vi "Dashboard Main.vi"() -> ()   [LabVIEW 2017]
uses:
  <vilib>/Rock Robotics/WPI/DriverStation/WPI_DriverStationAllianceInfo.ctl
  <vilib>/Utility/miscctls.llb/LVRowAndColumnTypeDef.ctl
  <vilib>/event_ctls.llb/eventvkey.ctl
  <vilib>/Rock Robotics/Network Tables/NT Read Numeric Array.vi
  <vilib>/Rock Robotics/WPI/Dashboard/WPI_DashboardLogging Global.vi
  <vilib>/Rock Robotics/Network Tables/NT Write Numeric Array.vi
  <vilib>/Rock Robotics/Network Tables/NT Read Boolean.vi
  <vilib>/Rock Robotics/Network Tables/NT Write Boolean.vi
panel:
  out "NT Connection":bool=TRUE
  in  "Camera Settings Right":T1={"Frame Rate"=15, "Compression"=30, "Size"=1, "DB Camera Config"=FALSE} {"Frame Rate" scale=1.0..30.0; "Compression" scale=100.0..-1.0; "Size" items=["640x480", "320x240", "160x120"]}
  in  "Camera Name Right":string(combo)="No Camera Selection"
  out "Camera Info":cluster{"Mbps LED":bool, "Mbps":dbl, "fps":dbl}={"Mbps LED"=FALSE, "Mbps"=0.17652911574406902, "fps"=9.930486593843098} {"fps" format="%#.1g"; "Mbps" format="%#.1g"}
  in  "Camera Settings":T1={"Frame Rate"=10, "Compression"=66, "Size"=2, "DB Camera Config"=FALSE} {"Frame Rate" scale=1.0..30.0; "Compression" scale=100.0..-1.0; "Size" items=["640x480", "320x240", "160x120"]}
  in  "TCP":refnum<k5>
  in  "Rec Mode":enum32{"Stop", "Record", "Playback"}(radio)
  out "Robot IP":string="10.17.12.2"
  out "Image Message":string="Timeout in Camera Communications"
  in  "Dashboard Tab":T2(tab)
  out "PixyX":dbl(slide)=26.65616755102041 scale=0.0..320.0
  in  "Reset":bool
  out "FastMode":bool
  out "ToggleMode":bool
  out "HasCube":bool
  out "Mode":T3(ring)
  out "Gyro":dbl(knob)=-172.57 scale=-180.0..180.0
  out "Elevator":dbl(slide)=5.727272727272727 scale=-10.0..80.0
  out "LeftEncoder":dbl=817.74403425
  out "RightEncoder":dbl=362.091195
  out "Ultrasonic":dbl(slide)=26.65616755102041 scale=0.0..60.0
  out "Bottom":bool
  out "Top":bool
  out "Camera Image Right":T4(plugin-control)
  in  "DB/String 9":string
  in  "DB/String 8":string
  in  "DB/String 7":string
  in  "DB/String 6":string
  in  "DB/String 5":string
  in  "DB/String 4":string
  in  "DB/String 3":string
  in  "DB/String 2":string
  in  "DB/String 1":string
  in  "DB/String 0":string
  in  "DB/Slider 0":dbl(slide) scale=0.0..5.0
  in  "DB/Slider 1":dbl(slide) scale=0.0..5.0
  in  "DB/Slider 2":dbl(slide) scale=0.0..5.0
  in  "DB/Slider 3":dbl(slide) scale=0.0..5.0
  out "DB/LED 3":bool
  out "DB/LED 2":bool
  out "DB/LED 1":bool
  out "DB/LED 0":bool
  in  "DB/Button 3":bool
  in  "DB/Button 2":bool
  in  "DB/Button 1":bool
  in  "DB/Button 0":bool caption="New Name"
  in  "RR Delay":dbl
  in  "LR Delay":dbl
  in  "LL Delay":dbl
  in  "RRAction2":dbl
  in  "LRAction2":dbl
  in  "LLAction2":dbl
  in  "RRAction1":dbl
  in  "LRAction1":dbl
  in  "LLAction1":dbl
  in  "NotPurePursuit":bool
  in  "Battery Number":string
  out "?":bool=TRUE
  out "Opponent Right Switch":bool
  out "Center Left Scale":bool=TRUE
  out "Center Right Scale":bool
  out "Our Left Team Switch":bool=TRUE
  out "Our Right Team Switch":bool
  in  "Position":u32=3
  in  "RLAction1":dbl
  in  "RLAction2":dbl
  in  "RL Delay":dbl
  in  "Test Slider":dbl(slide) scale=0.0..100.0 scale format="%#_3g"
  in  "On/Off":bool caption="Solenoid"
  in  "Test Name":u16(ring) items=["Select the test to run..."]
  in  "Test Tree":string(tree)
  in  "Motor":cluster{"Value":dbl, "Enable":bool} {"Value" scale=-1.0..1.0 scale format="%#_3g"}
  out "Progress":T5 {"Test Progress" scale=0.0..100.0}
  in  "Rev/Fwd":cluster{"Forward":bool, "Reverse":bool}
  in  "Test Ring":u16(ring) items=["Monochrome", "Color"]
  out "Cmd Status":string
  in  "Execute Command":bool
  in  "Command Params":string[][](table)
  in  "Command Selection":i32(listbox)
  in  "CheckList":i32(listbox)
  out "Tree":string(tree)
  out "Camera Image":T4(plugin-control)
  in  "Camera Name":string(combo)="Camera"
  # "Don't use this row"
  # "HW"
  # "HW"
  # "Switch/Scale Positions"
  # "1Cube"
  # "2Cube"
  # "Delay"
  # "Left"
  # "Left"
  # "Right"
  # "Left"
  # "Left"
  # "Right"
  # "Right"
  # "Right"
  # "Action Key:\n0 = Do Nothing\n1 = Go Switch\n2 = Go Scale"
  # "1"
  # "2"
  # "3"
  # "4"
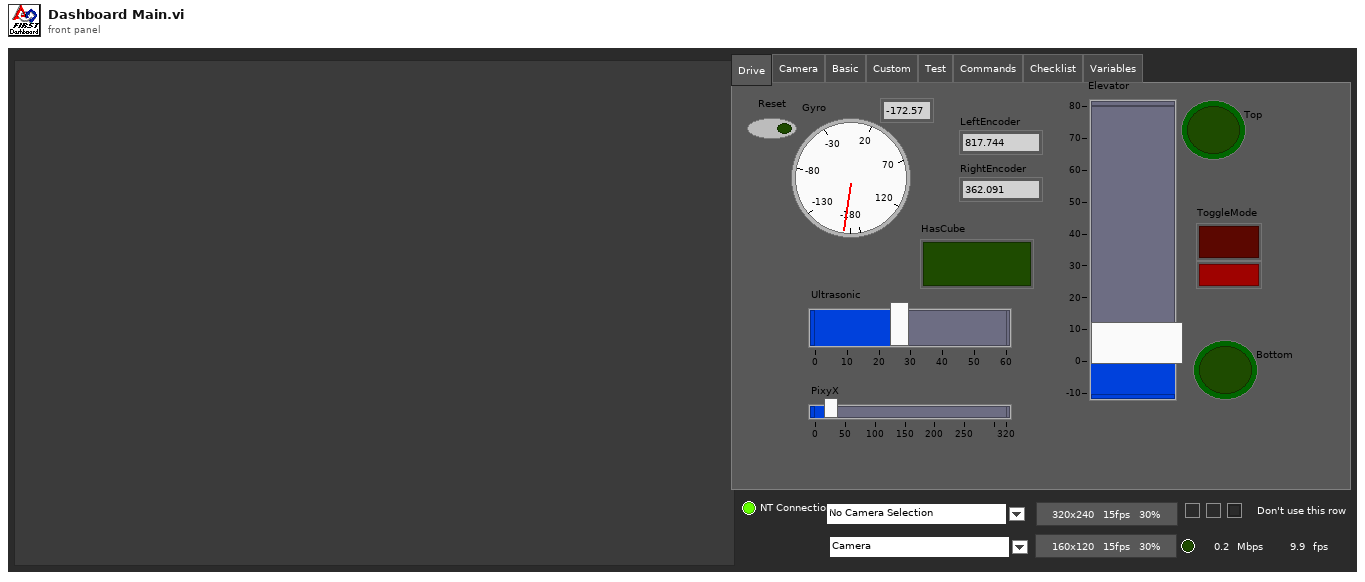
[diagram p1: front panel]
types:
  T1 = cluster{"Frame Rate":i32, "Compression":i32, "Size":u16, "DB Camera Config":bool}
  T2 = enum32{"Drive", "Camera", "Basic", "Custom", "Test", "Commands", "Checklist", "Variables"}
  T3 = enum8{"Tele-Op Disabled", "Tele-Op Enabled", "Auto Disabled", "Auto Enabled", "Test Disabled", "Test Enabled", "Disconnected", "No Code", "E-Stop"}
  T4 = typedef "IMAQ Image.ctl" = refnum<image>
  T5 = cluster{"Test Progress":u8, "Test Progress Text":string}
  T6 = cluster{"Save Path":path, "Interval (s)":dbl, "Keep":i32}
  T7 = typedef "Image Type" = u32
  T8 = cluster{"IDs":cluster{"RPC field ID":u16, "Unique ID":u16}, "String":string}
  T9 = cluster{"Error Strings":string, "Disable Counts":cluster{u16, u16}, "Rail Faults":cluster{u16, u16, u16}, "Robot IP":string, "DB Mode":u8, "Event Info":cluster{"Name":string, "Type":u8, "Number":u16, "Replay":u8}}
  T10 = cluster{"Storage":cluster{"Disk Free":u64, "RAM Block":u32, "RAM free":u32}, "CPU Utilization":cluster{"CPU % ISR":sgl, "CPU % Time Crit":sgl, "CPU % Timed Str":sgl, "CPU % High":sgl, "CPU % Above":sgl, "CPU % Normal":sgl, "CPU % Low":sgl}, "CAN":cluster{"% Bus Utilization":sgl, "Bus Off Cnt":u32, "TX_FIFO Full Cnt":u32, "Receive Error Cnt":u8, "Transmit Error Cnt":u8}, "HID":cluster{"HID Outputs":u32, "Rumble Low":u16, "Rumble High":u16}[]}
  T11 = cluster{"Status bits":cluster{"Test Mode":bool, "Autonomous":bool, "Enabled":bool, "Code Start":bool, "Brownout":bool, "Reserved 2":bool, "Reserved 3":bool, "E-Stop":bool}, "Code Trace":cluster{"Disabled":bool, "TeleOp":bool, "Auto":bool, "Test":bool}, "Controller Type":enum16{"unknown", "cRIO", "roboRio"}, "Code?":enum16{"unknown", "noCode", "code"}, "Battery V":dbl}
  T12 = cluster{"Control Bits":cluster{"TestMode":bool, "Autonomous":bool, "Enabled":bool, "FMS Present":bool, bool, bool, bool, "E-Stop":bool}, "Team Station ":u8, "Countdown":sgl, "Joystick Values":cluster{"Axes":dbl[], "Buttons":bool[], "POVs":i16[]}[]}
  T13 = cluster{"Axes":dbl[], "Buttons":bool[], "POVs":i16[]}[]
  T14 = cluster{"Axes":dbl[], "Buttons":bool[], "POVs":i16[]}
  T15 = cluster{"Camera Image":refnum<vi>, "Dashboard Tab":refnum<vi>, "Rec Mode":refnum<vi>, "Test Slider":refnum<vi>, "On/Off ":refnum<vi>, "Test Ring":refnum<vi>, "Rev/Fwd":refnum<vi>, "Test Name":refnum<vi>, "Motor":refnum<vi>, "Progress":refnum<vi>, "CheckList":refnum<vi>, "Tree":refnum<vi>, "Test Tree":refnum<vi>, "Command Params":refnum<vi>, "Command Selection":refnum<vi>, "Execute Command":refnum<vi>, "Cmd Status":refnum<vi>, "Camera Settings":refnum<vi>, "Camera Name":refnum<vi>, "Camera Info":refnum<vi>, "Camera Settings Right":refnum<vi>, "Camera Name Right":refnum<vi>, "Camera Image Right":refnum<vi>}
  T16 = cluster{"Camera Name":string, string, "Saved DB Images Info":cluster{"Save Path":path, "Interval (s)":dbl, "Keep":i32}}
  T17 = cluster{"Camera Name Right":string, string, "Saved DB Images Info":cluster{"Save Path":path, "Interval (s)":dbl, "Keep":i32}}
  T18 = typedef "WPI_DriverStationAllianceInfo.ctl" = enum16{"Red", "Blue", "Invalid"}
  T19 = cluster{"Operation":enum16{"Update", "Clear"}, "Color Box":u32}[]
  T20 = typedef "eventvkey.ctl" = enum16{"ASCII", "Enter", "Return", "Shift", "Ctrl", "Alt", "Cmd", "Opt", "Caps", "NumLock", "Clear", "Break", "Up", "Down", "Left", "Right", "Insert", "Delete", "Home", "End", "PageUp", "PageDown", "Escape", "Help", "Pause", "ScrollLock", "F1", "F2", "F3", "F4", "F5", "F6", "F7", "F8", "F9", "F10", "F11", "F12", "F13", "F14", "F15", "F16", "F17", "F18", "F19", "F20", "F21", "F22", "F23", "F24", "Play", "VolumeUp", "VolumeDown", "Mute", "Two Byte Char"}
  T21 = cluster{"Image Size":bool, "Image Type":bool, "Pixel Value":bool, "ROI Information":bool, "Zoom Factor":bool}
  T22 = cluster{"Operation":enum16{"Update", "Clear"}, "Color Box":u32}
  T23 = typedef "LVRowAndColumnTypeDef.ctl" = cluster{"Row":i32, "Column":i32}
  T24 = cluster{"Shift":bool, "Ctrl":bool, "Alt":bool, "Cmd":bool, "Opt":bool}
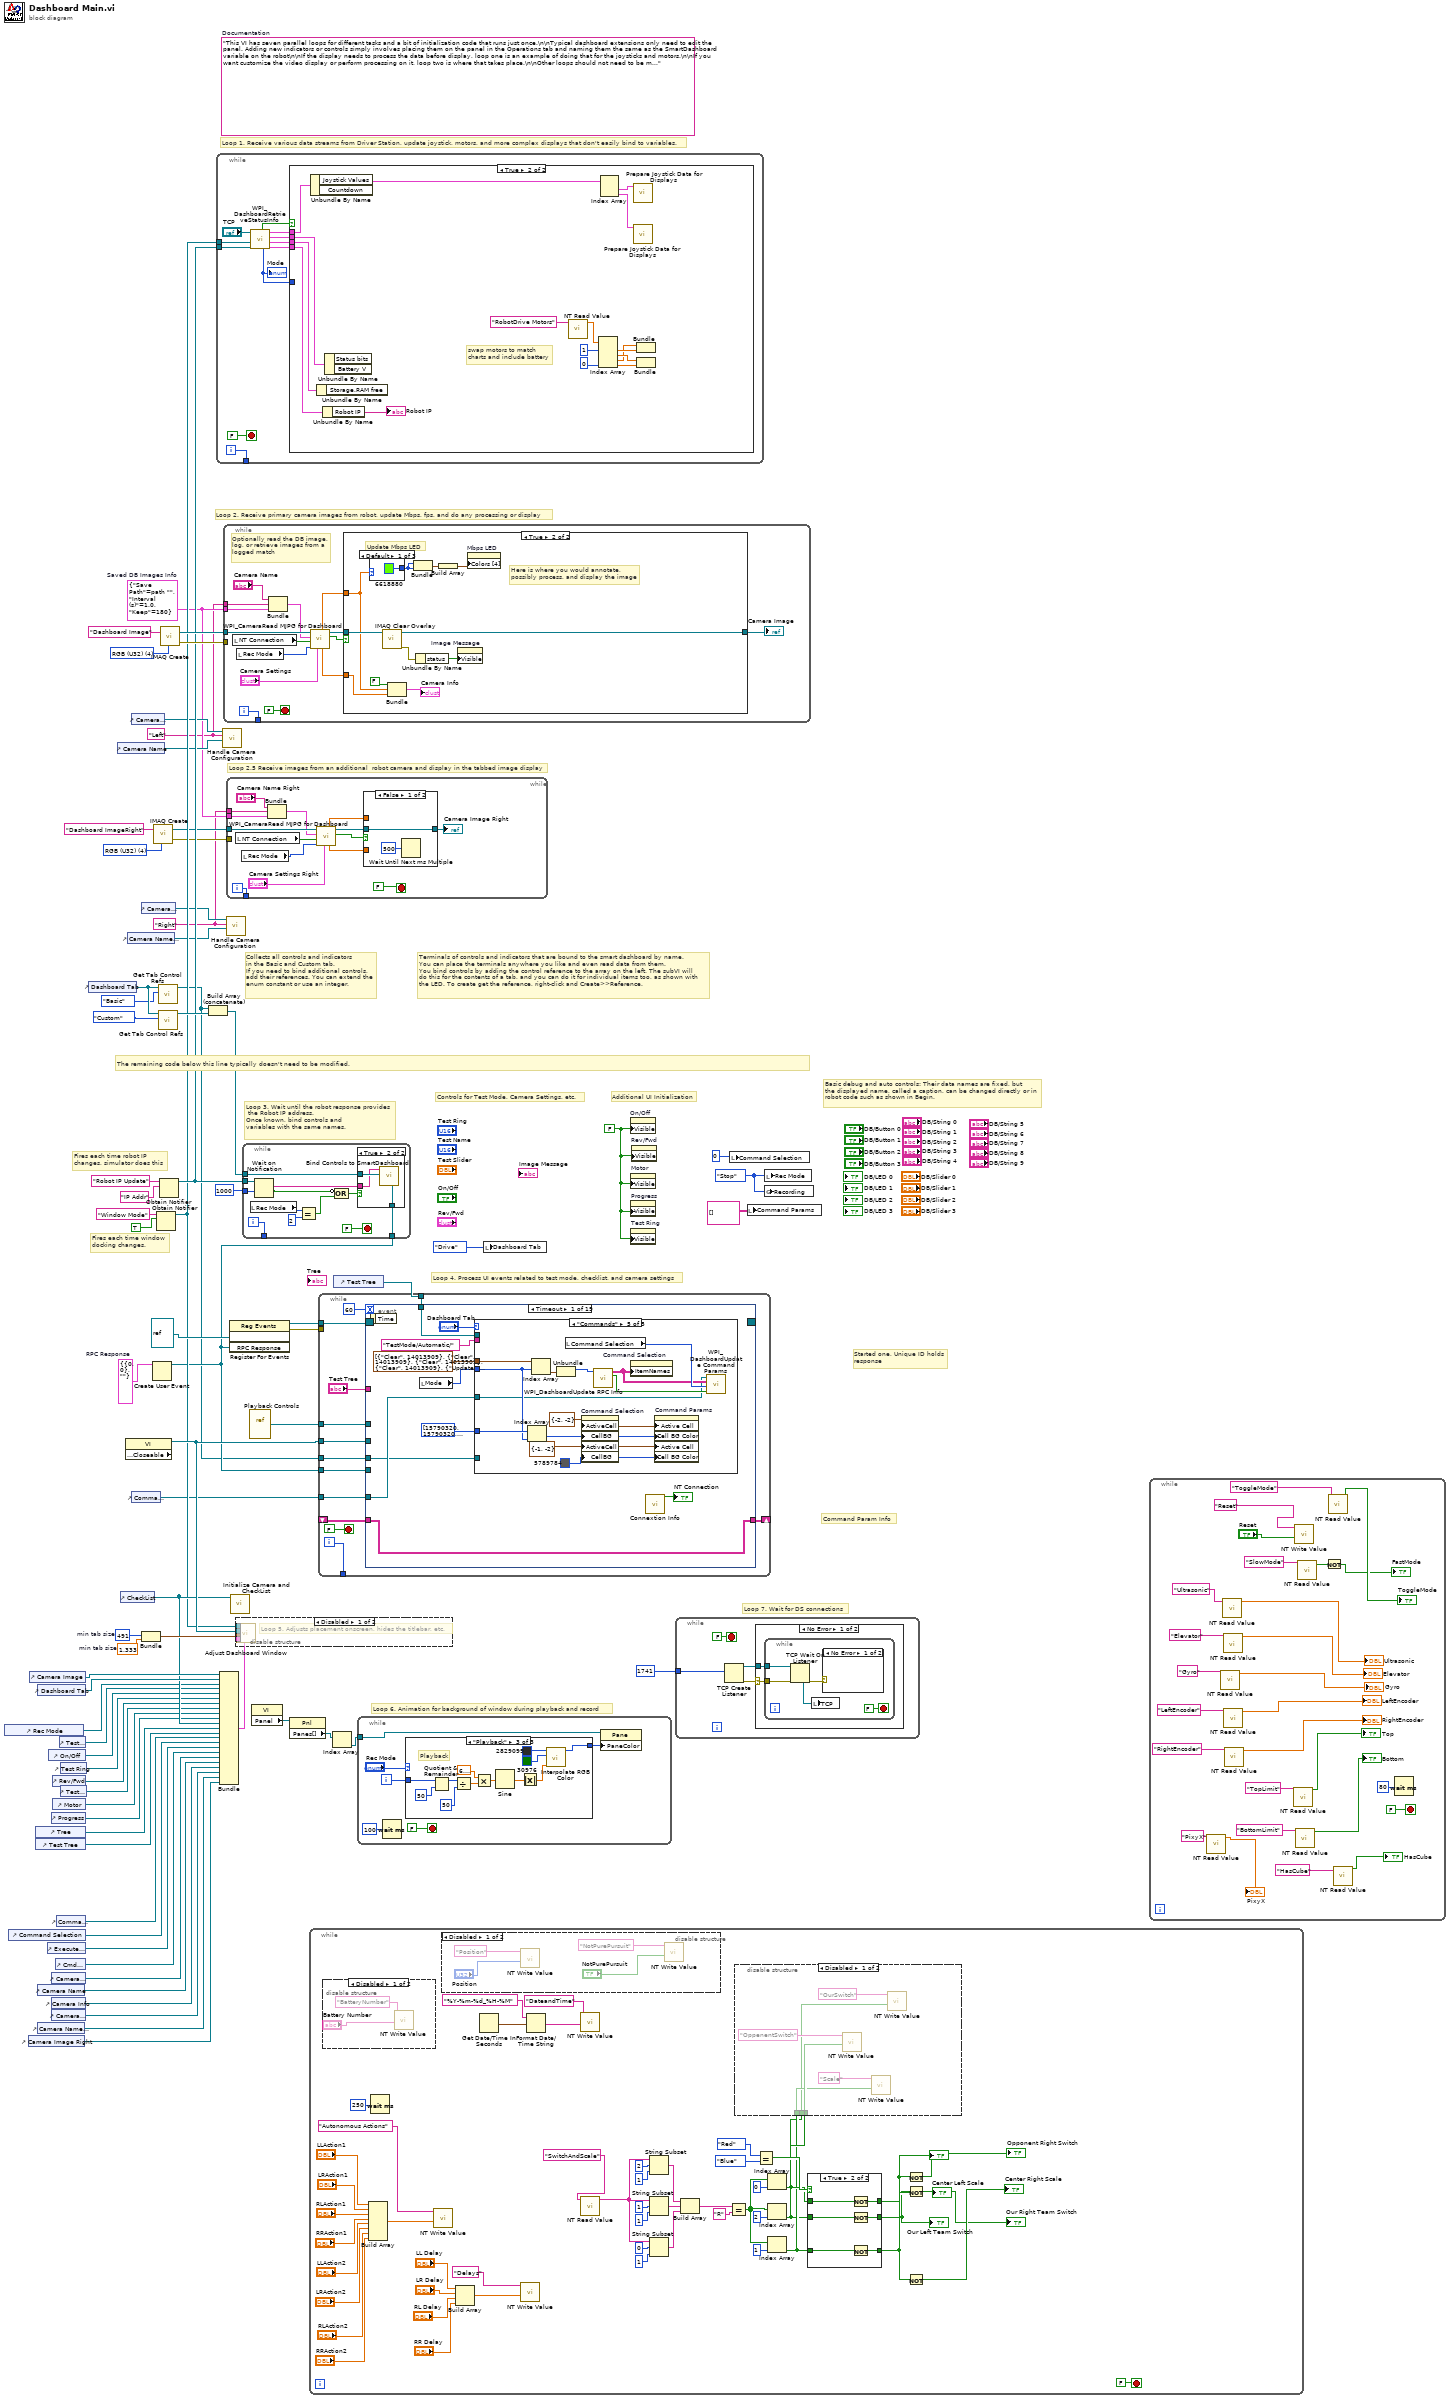
[diagram p0: block diagram]
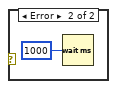
[diagram p8: hidden frame]
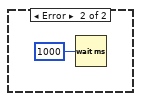
[diagram p9: hidden frame]
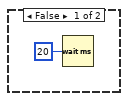
[diagram p10: hidden frame]
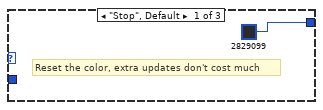
[diagram p11: hidden frame]
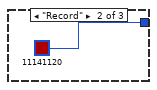
[diagram p12: hidden frame]
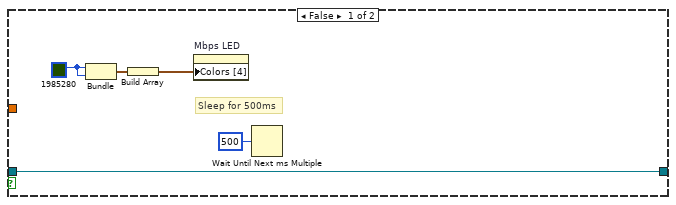
[diagram p14: hidden frame]
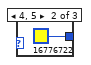
[diagram p15: hidden frame]
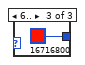
[diagram p16: hidden frame]
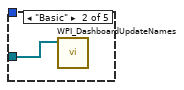
[diagram p18: hidden frame]
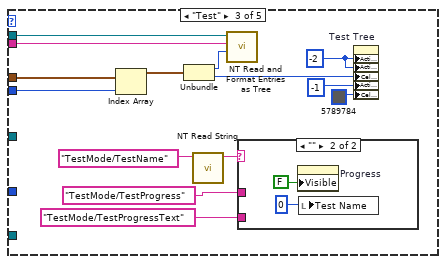
[diagram p19: hidden frame]
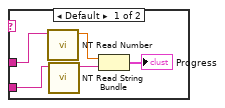
[diagram p20: hidden frame]
diagram:
  w4 = T6 {"Save Path"=path "", "Interval (s)"=1.0, "Keep"=180}  # Saved DB Images Info
  w3 = "Right"
  w2 = "Left"
  w14 = T7 4 items=["Grayscale (U8)", "Grayscale (I16)", "Grayscale (SGL)", "Complex (CSG)", "RGB (U32)", "HSL (U32)", "RGB (U64)"] ("Image Type")
  w28 = T8 {"IDs"={"RPC field ID"=0, "Unique ID"=0}, "String"=""}  # RPC Response
  w49 = 491  # min tab size
  w48 = 1.333  # min tab size
  w56 = enum32{"Stop", "Record", "Playback"}."Stop" ("Rec Mode")
  w34 = FALSE ("Visible")
  (unwired) "This VI has seven parallel loops for different tasks and a bit of initialization code that runs just once.\n\nTypical dashboard extensions only need to edit the panel. Adding new indicators or controls simply involves placing them on the panel in the Operations tab and naming them the same as the SmartDashboard variable on the robot\n\nIf the display needs to process the data before display, loop one is an example of doing that for the joysticks and motors.\n\nIf you want customize the video display or perform processing on it, loop two is where that takes place.\n\nOther loops should not need to be modified. They are pretty standard, and document the task they perform."  # Documentation
  w73 = T7 4 items=["Grayscale (U8)", "Grayscale (I16)", "Grayscale (SGL)", "Complex (CSG)", "RGB (U32)", "HSL (U32)", "RGB (U64)"] ("Image Type")
  # "Loop 2.5 Receive images from an additional  robot camera and display in the tabbed image display"
  # "Command Param Info"
  # "Started one, Unique ID holds\nresponse"
  # "Loop 7. Wait for DS connections"
  # "Basic debug and auto controls: Their data names are fixed, but\nthe displayed name, called a caption, can be changed directly or in\nrobot code such as shown in Begin."
  # "Controls for Test Mode, Camera Settings, etc."
  # "Additional UI Initialization"
  # "Loop 6. Animation for background of window during playback and record"
  # "Fires each time robot IP\nchanges, simulator does this"
  # "Fires each time window\ndocking changes."
  # "Collects all controls and indicators\nin the Basic and Custom tab.\nIf you need to bind additional controls,\nadd their references. You can extend the\nenum constant or use an integer."
  # "The remaining code below this line typically doesn't need to be modified."
  # "Loop 4. Process UI events related to test mode, checklist, and camera settings"
  # "Terminals of controls and indicators that are bound to the smart dashboard by name.\nYou can place the terminals anywhere you like and even read data from them.\nYou bind controls by adding the control reference to the array on the left. The subVI will\ndo this for the contents of a tab, and you can do it for individual items too, as shown with\nthe LED. To create get the reference, right-click and Create>>Reference."
  # "Loop 3. Wait until the robot response provides\n the Robot IP address.\nOnce known, bind controls and\nvariables with the same names."
  # "Loop 1. Receive various data streams from Driver Station, update joystick, motors, and more complex displays that don't easily bind to variables."
  # "Loop 2. Receive primary camera images from robot, update Mbps, fps, and do any processing or display"
  n1 = control-ref of="Rec Mode"() -> (w40:refnum<vi>)
  n2 = control-ref of="Command Selection"() -> (w27:refnum<vi>)
  n3 = control-ref of="Camera Image Right"() -> (w7:refnum<vi>)
  n4 = control-ref of="Camera Image"() -> (w51:refnum<vi>)
  n5 = control-ref of="Tree"() -> (w44:refnum<vi>)
  n6 = control-ref of="Test Tree"() -> (w43:refnum<vi>)
  n7 = control-ref of="Dashboard Tab"() -> (w50:refnum<vi>)
  n8 = control-ref of="Camera Name"() -> (w18:refnum<vi>)
  n9 = control-ref of="Camera Name Right"() -> (w8:refnum<vi>)
  n10 = control-ref of="Execute Command"() -> (w29:refnum<vi>)
  n11 = control-ref of="On/Off"() -> (w38:refnum<vi>)
  n12 = control-ref of="Progress"() -> (w35:refnum<vi>)
  n13 = control-ref of="Camera Settings"() -> (w19:refnum<vi>)
  n14 = control-ref of="Camera Info"() -> (w17:refnum<vi>)
  n15 = control-ref of="Camera Settings Right"() -> (w9:refnum<vi>)
  n16 = control-ref of="Rev/Fwd"() -> (w36:refnum<vi>)
  n17 = control-ref of="Motor"() -> (w41:refnum<vi>)
  n18 = control-ref of="Cmd Status"() -> (w23:refnum<vi>)
  n19 = control-ref of="Command Params"() -> (w30:refnum<vi>)
  n20 = control-ref of="Test Slider"() -> (w39:refnum<vi>)
  n21 = control-ref of="Test Ring"() -> (w37:refnum<vi>)
  n22 = control-ref of="Test Name"() -> (w42:refnum<vi>)
  n23 = control-ref of="Dashboard Tab"() -> (w54:refnum<vi>)
  n24 = control-ref of="Camera Name"() -> (w20:refnum<vi>)
  n25 = control-ref of="CheckList"() -> (w45:refnum<vi>)
  n26 = property class="VI" props=["Front Panel.Closeable"]() -> (reference out=w55:refnum<vi>)  [unwired: 2 in, 2 out]
  n27 = control-ref of="Camera Name Right"() -> (w10:refnum<vi>)
  n28 = control-ref of="Camera Settings"() -> (w21:refnum<vi>)
  n29 = control-ref of="Command Params"() -> (w22:refnum<vi>)
  n30 = control-ref of="Camera Settings Right"() -> (w11:refnum<vi>)
  n31 = Bundle("min tab size"=w49, "min tab size"=w48) -> (w47:cluster{"min tab size":i32, "min tab size":dbl})  [unwired: 1 in]
  n32 = Create User Event(user event datatype=w28) -> (user event=w24:refnum<user-event>)  [unwired: 1 in, 1 out]
  n33 = call "IMAQ Create"("Image Name"="Dashboard ImageRight", "Image Type"=w14) -> ("New Image"=w13:T4, "error out"=w12:errorcluster)  [unwired: 2 in, 1 out]
  n34 = Obtain Notifier(name (unnamed)="Window Mode", notification data type=TRUE) -> (notifier out=w32:refnum<notifier>)  [unwired: 2 in, 2 out]
  n35 = call <vilib>:"Get Tab Control Refs.vi"("Page Index"=T2."Basic" ("Dashboard Tab"), "TabControl in"=w54) -> ("ControlsOnPage"=w16:refnum<vi>[])  [unwired: 9 in]
  n36 = call <vilib>:"Get Tab Control Refs.vi"("Page Index"=T2."Custom" ("Dashboard Tab"), "TabControl in"=w54) -> ("ControlsOnPage"=w53:refnum<vi>[])  [unwired: 9 in]
  n37 = Obtain Notifier(name (unnamed)="Robot IP Update", notification data type="IP Addr" ("name (unnamed)")) -> (notifier out=w33:refnum<notifier>)  [unwired: 2 in, 2 out]
  n38 = call "IMAQ Create"("Image Name"="Dashboard Image", "Image Type"=w73) -> ("New Image"=w71:T4, "error out"=w70:errorcluster)  [unwired: 2 in, 1 out]
  n39 = Build Array (concatenate)(w16, w53) -> (w52:refnum<vi>[])
  n40 = while {
    tunnel: [w83] -> _
    tunnel: w33 -> [w77]
    tunnel: w32 -> [w74]
    i -> [w83]
    stop <- FALSE stop-if-true
    n41 = call <vilib>:"WPI_DashboardRetrieveStatusInfo.vi"("Binding Refnum"=w77, "Window Mode Notifier"=w74, "TCP Cnx"="TCP") -> ("Power and Errors"=w78:T9, "Robot Metrics"=w81:T10, "Status Info"=w82:T11, "Control Info"=w79:T12, "Robot Mode"=w76:T3, "Process?"=w80:bool)  [unwired: 3 in]
    "Mode" <- w76
    n42 = case shown="True" w80 {
      tunnel: w82 -> [_ w101]
      tunnel: w81 -> [_ w100]
      tunnel: w79 -> [_ w99]
      tunnel: w78 -> [_ w98]
      tunnel: w76 -> [_ _]
      frame False {
        n43 = Wait (ms)(milliseconds to wait=u32 20) -> ()  [unwired: 1 out]
      }
      frame True {
        # "swap motors to match\ncharts and include battery"
        n44 = Unbundle By Name(w99) -> ("Joystick Values"=w91:T13)  [unwired: 1 out]
        n45 = Unbundle By Name(w100) -> ()  [unwired: 1 out]
        n46 = Unbundle By Name(w98) -> ("Robot IP"=→"Robot IP":string)
        n47 = Unbundle By Name(w101) -> ()  [unwired: 2 out]
        n48 = call-poly <vilib>:"NT Read Value.vi"("Name"="RobotDrive Motors") -> ("Numeric Array"=w87:dbl[])  [unwired: 9 in, 1 out]
        n49 = Index Array(array=w87, index #1=1, index #4=0) -> (element #1=w93:dbl, element #2=w94:dbl, element #3=w92:dbl, element #4=w97:dbl)  [unwired: 2 in]
        n50 = Index Array(array=w91) -> (element #1=w90:T14, element #2=w89:T14)  [unwired: 2 in]
        n51 = call "Prepare Joystick Data for Displays.vi"("Joystick Values"=w89) -> ()  [unwired: 8 in, 3 out]
        n52 = call "Prepare Joystick Data for Displays.vi"("Joystick Values"=w90) -> ()  [unwired: 8 in, 3 out]
        n53 = Bundle("Numeric"=w92, "Numeric"=w93) -> ()  [unwired: 1 in, 1 out]
        n54 = Bundle("Numeric"=w94, "Numeric"=w97) -> ()  [unwired: 1 in, 1 out]
      }
    }
  }
  n55 = Bundle("Camera Image"=w51, "Dashboard Tab"=w50, "Rec Mode"=w40, "Test Slider"=w39, "On/Off"=w38, "Test Ring"=w37, "Rev/Fwd"=w36, "Test Name"=w42, "Motor"=w41, "Progress"=w35, "CheckList"=w45, "Tree"=w44, "Test Tree"=w43, "Command Params"=w30, "Command Selection"=w27, "Execute Command"=w29, "Cmd Status"=w23, "Camera Settings"=w19, "Camera Name"=w18, "Camera Info"=w17, "Camera Settings Right"=w9, "Camera Name Right"=w8, "Camera Image Right"=w7) -> (w46:T15)  [unwired: 1 in]
  n56 = call "Handle Camera Configuration.vi"("CameraNameRef"=w20, "Display Name"=w2, "ClusterRef"=w21) -> ()  [unwired: 9 in]
  n57 = while {
    tunnel: w71 -> [w114]
    tunnel: w70 -> [_]
    tunnel: [w115] -> _
    tunnel: w4 -> [w105]
    tunnel: w2 -> [w102]
    i -> [w115]
    stop <- FALSE stop-if-true
    # "Optionally read the DB image,\nlog, or retrieve images from a\nlogged match"
    n58 = local read "NT Connection"() -> (w106:bool)
    n59 = local read "Rec Mode"() -> (w110:enum32{"Stop", "Record", "Playback"})
    n60 = Bundle("Camera Name"="Camera Name", w102, "Saved DB Images Info"=w105) -> (w104:T16)  [unwired: 1 in]
    n61 = call <vilib>:"WPI_CameraRead MJPG for Dashboard.vi"("Camera Settings"="Camera Settings", "Rec Mode"=w110, "NT Connection"=w106, "Capture Info"=w104, "Refnum in"=w114) -> ("Active"=w112:bool, "Refnum out"=w113:T4, "FPS"=w111:dbl, "Bandwidth (Mbps)"=w109:dbl)  [unwired: 3 in]
    n62 = case shown="True" w112 {
      tunnel: w113 -> [w117 w128]
      tunnel: w109 -> [_ w125]
      tunnel: w111 -> [_ w126]
      tunnel: [w117 w122] -> w107
      frame False {
        w119 = u32 1985280 ("Color Box")
        # "Sleep for 500ms"
        n63 = Bundle("Color Box"=w119, "Color Box"=w119) -> (w120:cluster{"Color Box":u32, "Color Box":u32})  [unwired: 1 out]
        n64 = Build Array(w120) -> (w118:cluster{"Color Box":u32, "Color Box":u32}[])
        n65 = property on="Mbps LED" class="Bool (strict)"("Colors [4]"=w118) -> ()  [unwired: 2 in, 2 out]
        n66 = Wait Until Next ms Multiple(millisecond multiple=u32 500) -> ()  [unwired: 1 out]
      }
      frame True {
        # "Here is where you would annotate,\npossibly process, and display the image"
        # "Update Mbps LED"
        n67 = case shown="Default" w125 {
          tunnel: [u32 6618880 ("Color Box") u32 16776722 ("Color Box") u32 16716800 ("Color Box")] -> w129
          frame Default {
          }
          frame 4, 5 {
          }
          frame 6.. {
          }
        }
        n68 = call "IMAQ Clear Overlay"("Image"=w128) -> ("error out"=w131:errorcluster, "Image Out"=w122:T4)  [unwired: 2 in, 7 out]
        n69 = Bundle(FALSE, "Bandwidth (Mbps)"=w125, "FPS"=w126) -> (→"Camera Info":cluster{bool, "Bandwidth (Mbps)":dbl, "FPS":dbl})  [unwired: 1 in]
        n70 = Bundle("Color Box"=w129, "Color Box"=w129) -> (w130:cluster{"Color Box":u32, "Color Box":u32})  [unwired: 1 out]
        n71 = Unbundle By Name(w131) -> ("status"=w132:bool)
        n72 = Build Array(w130) -> (w127:cluster{"Color Box":u32, "Color Box":u32}[])
        n73 = property on="Image Message" class="Str"("Visible"=w132) -> ()  [unwired: 2 in, 2 out]
        n74 = property on="Mbps LED" class="Bool (strict)"("Colors [4]"=w127) -> ()  [unwired: 2 in, 2 out]
      }
    }
    "Camera Image" <- w107
  }
  n75 = call "Handle Camera Configuration.vi"("CameraNameRef"=w10, "Display Name"=w3, "ClusterRef"=w11) -> ()  [unwired: 9 in]
  n76 = while {
    tunnel: w13 -> [w150]
    tunnel: w12 -> [_]
    tunnel: [w145] -> _
    tunnel: w4 -> [w139]
    tunnel: w3 -> [w136]
    i -> [w145]
    stop <- FALSE stop-if-true
    n77 = local read "NT Connection"() -> (w140:bool)
    n78 = local read "Rec Mode"() -> (w149:enum32{"Stop", "Record", "Playback"})
    n79 = Bundle("Camera Name Right"="Camera Name Right", w136, "Saved DB Images Info"=w139) -> (w138:T17)  [unwired: 1 in]
    n80 = call <vilib>:"WPI_CameraRead MJPG for Dashboard.vi"("Camera Settings"="Camera Settings Right", "Rec Mode"=w149, "NT Connection"=w140, "Capture Info"=w138, "Refnum in"=w150) -> ("Active"=w144:bool, "Refnum out"=w147:T4, "FPS"=w142:dbl, "Bandwidth (Mbps)"=w143:dbl)  [unwired: 3 in]
    n81 = case shown="False" w144 {
      tunnel: w147 -> [w151 w153]
      tunnel: w143 -> [_ _]
      tunnel: w142 -> [_ _]
      tunnel: [w151 w153] -> w141
      frame False {
        n82 = Wait Until Next ms Multiple(millisecond multiple=u32 500) -> ()  [unwired: 1 out]
      }
      frame True {
      }
    }
    "Camera Image Right" <- w141
  }
  n83 = register-events(refnum<vi> refnum, w24) -> (reference out=w60:refnum<event-registration>, error out=w59:errorcluster)  [unwired: 2 in]
  n84 = call "Initialize Camera and CheckList.vi"("ListBox in"=w45) -> ()  [unwired: 11 in]
  n85 = disable-structure shown="Disabled" {
    disable-tunnel: w55 -> [w157 _]
    disable-tunnel: w47 -> [w156 _]
    disable-tunnel: w46 -> [w155 _]
    disable-tunnel: w32 -> [w154 _]
    frame Disabled {
      # "Loop 5. Adjusts placement onscreen, hides the titlebar, etc."
      n86 = call "Adjust Dashboard Window.vi"("Sizing Refnums"=w155, "Size Constraints"=w156, "VI"=w157, "WIn Mode"=w154) -> ()  [unwired: 8 in]
    }
    frame Enabled {
    }
  }
  n87 = while {
    tunnel: w52 -> [w169]
    tunnel: w33 -> [w167]
    tunnel: [w165] -> _
    tunnel: u32 1000 ("milliseconds to wait") -> [w164]
    tunnel: w24 -> [w158]
    i -> [w165]
    stop <- FALSE stop-if-true
    n88 = local read "Rec Mode"() -> (w160:enum32{"Stop", "Record", "Playback"})
    n89 = Wait on Notification(notifier=w167, timeout in ms (-1)=w164) -> (notification=w166:string, timed out?=w162:bool)  [unwired: 2 in, 2 out]
    n90 = Equal?(x=w160, y=u16 2 ("Rec Mode")) -> (x = y?=w161:bool)
    n91 = Compound Arithmetic op=OR(invert w162, w161) -> (w163:bool)
    n92 = case shown="True" w163 {
      tunnel: w169 -> [_ w172]
      tunnel: w166 -> [_ w171]
      tunnel: w158 -> [_ w170]
      frame False {
      }
      frame True {
        n93 = call <vilib>:"Bind Controls to SmartDashboard.vi"("RPC ref"=w170, "Bound Control Refs"=w172, "Server IP Address"=w171) -> ()  [unwired: 9 in]
      }
    }
  }
  n94 = vi-ref "Playback Controls.vi"() -> (w61:refnum<vi>)
  n95 = property class="VI"() -> ("Panel"=w63:refnum<vi>)  [unwired: 2 in, 2 out]
  n96 = property class="Pnl"(reference=w63) -> ("Panes[]"=w64:refnum<vi>[])  [unwired: 1 in, 2 out]
  n97 = while {
    stop <- FALSE stop-if-true
    n98 = disable-structure shown="Disabled" {
      frame Disabled {
        n99 = call-poly <vilib>:"NT Write Value.vi"("String"="Battery Number", "Name"="BatteryNumber") -> ()  [unwired: 9 in, 1 out]
      }
      frame Enabled {
      }
    }
    n100 = Build Array("LLAction1", "LRAction1", "RLAction1", "RRAction1", "LLAction2", "LRAction2", "RLAction2", "RRAction2") -> (w183:dbl[])
    n101 = Wait (ms)(milliseconds to wait=u32 250) -> ()  [unwired: 1 out]
    n102 = call-poly <vilib>:"NT Write Value.vi"("Numeric Array"=w183, "Name"="Autonomous Actions") -> ()  [unwired: 9 in, 1 out]
    n103 = disable-structure shown="Disabled" {
      frame Disabled {
        n104 = call-poly <vilib>:"NT Write Value.vi"("Numeric"="Position", "Name"="Position") -> ()  [unwired: 9 in, 1 out]
        n105 = call-poly <vilib>:"NT Write Value.vi"("Boolean"="NotPurePursuit", "Name"="NotPurePursuit") -> ()  [unwired: 9 in, 1 out]
      }
      frame Enabled {
      }
    }
    n106 = Build Array("LL Delay", "LR Delay", "RL Delay", "RR Delay") -> (w179:dbl[])
    n107 = Get Date/Time In Seconds() -> (seconds since 1Jan1904=w220:timestamp)
    n108 = call-poly <vilib>:"NT Write Value.vi"("Numeric Array"=w179, "Name"="Delays") -> ()  [unwired: 9 in, 1 out]
    n109 = Format Date/Time String(time format string (%c)="%Y-%m-%d_%H-%M", seconds (now)=w220) -> (date/time string=w219:string)  [unwired: 1 in]
    n110 = call-poly <vilib>:"NT Write Value.vi"("String"=w219, "Name"="DateandTime") -> ()  [unwired: 9 in, 1 out]
    n111 = call-poly <vilib>:"NT Read Value.vi"("Name"="SwitchAndScale") -> ("String"=w191:string)  [unwired: 9 in, 1 out]
    n112 = String Subset(string=w191, offset (0)=2, length (rest)=1 ("length (rest)")) -> (substring=w213:string)
    n113 = String Subset(string=w191, offset (0)=1, length (rest)=1 ("length (rest)")) -> (substring=w212:string)
    n114 = String Subset(string=w191, offset (0)=0, length (rest)=1 ("length (rest)")) -> (substring=w211:string)
    n115 = Build Array(w213, w212, w211) -> (w210:string[])
    n116 = Equal?(x=w210, y="R") -> (x = y?=w205:bool[])
    n117 = Equal?(x=WPI_DriverStationAllianceInfo."Red" ("y"), y=WPI_DriverStationAllianceInfo."Blue") -> (x = y?=w201:bool)
    n118 = Index Array(array=w205, index=0) -> (element=w194:bool)
    n119 = Index Array(array=w205, index=2) -> (element=w192:bool)
    n120 = Index Array(array=w205, index=1) -> (element=w193:bool)
    n121 = disable-structure shown="Disabled" {
      disable-tunnel: w194 -> [w232 _]
      disable-tunnel: w193 -> [w231 _]
      disable-tunnel: w192 -> [w230 _]
      frame Disabled {
        n122 = call-poly <vilib>:"NT Write Value.vi"("Boolean"=w232, "Name"="OppenentSwitch") -> ()  [unwired: 9 in, 1 out]
        n123 = call-poly <vilib>:"NT Write Value.vi"("Boolean"=w231, "Name"="Scale") -> ()  [unwired: 9 in, 1 out]
        n124 = call-poly <vilib>:"NT Write Value.vi"("Boolean"=w230, "Name"="OurSwitch") -> ()  [unwired: 9 in, 1 out]
      }
      frame Enabled {
      }
    }
    n125 = case shown="True" w201 {
      tunnel: w192 -> [w236 w240]
      tunnel: [w236 w239] -> w196
      tunnel: w193 -> [w238 w242]
      tunnel: [w238 w241] -> w199
      tunnel: w194 -> [w237 w244]
      tunnel: [w237 w243] -> w197
      frame False {
      }
      frame True {
        n126 = Not(x=w244) -> (.not. x?=w243:bool)
        n127 = Not(x=w240) -> (.not. x?=w239:bool)
        n128 = Not(x=w242) -> (.not. x?=w241:bool)
      }
    }
    "?" <- w197
    "Center Left Scale" <- w199
    "Our Left Team Switch" <- w196
    n129 = Not(x=w197) -> (.not. x?=→"Opponent Right Switch":bool)
    n130 = Not(x=w196) -> (.not. x?=→"Our Right Team Switch":bool)
    n131 = Not(x=w199) -> (.not. x?=→"Center Right Scale":bool)
  }
  n132 = Index Array(array=w64) -> (element=w62:refnum<vi>)  [unwired: 1 in]
  n133 = control-ref of="Test Tree"() -> (w65:refnum<vi>)
  n134 = while {
    tunnel: [w254] -> _
    tunnel: w65 -> [w253]
    tunnel: w61 -> [w252]
    tunnel: w60 -> [w251]
    tunnel: w59 -> [_]
    tunnel: w55 -> [w250]
    tunnel: w24 -> [w249]
    tunnel: w22 -> [w248]
    shift-right: [w247] -> _
    shift-left: _ -> [w246]
    tunnel: w16 -> [w245]
    i -> [w254]
    stop <- FALSE stop-if-true
    n135 = event shown="[0] Timeout" {
      selector: w251 -> [_ _ _ _ _ _ _ _ _ _ _ _ _ _ _ _ _ _ _]
      dyn-events: [_ _ _ _ _ _ _ _ _ _ _ _ _ _ w508 _ _ _ _] -> _
      timeout: u32 60 ("milliseconds to wait") -> [_ _ _ _ _ _ _ _ _ _ _ _ _ _ _ _ _ _ _]
      tunnel: w253 -> [w266 _ _ _ _ _ _ _ _ _ _ _ _ _ _ _ _ _ _]
      tunnel: "Test Tree" -> [_ _ _ _ _ _ _ _ _ w475 w483 w485 w489 w497 _ _ _ _ _]
      tunnel: w252 -> [_ _ _ _ _ _ _ _ _ _ _ _ _ _ w510 _ w528 _ _]
      tunnel: w250 -> [_ _ _ _ _ _ _ _ _ _ _ _ _ _ w506 _ _ _ _]
      tunnel: w249 -> [_ _ _ _ _ _ _ _ _ _ _ _ _ _ w504 _ _ _ _]
      tunnel: w248 -> [w261 _ _ _ w426 _ _ _ _ _ _ _ _ _ _ _ _ _ _]
      tunnel: [w260 w309 w411 w416 w424 w433 w443 w450 w462 w474 w481 w484 w488 w496 w503 w523 w525 w529 w542] -> w247
      tunnel: w246 -> [w260 w309 w411 w416 w424 _ _ w450 w462 w474 w481 w484 w488 w496 w503 w523 w525 w529 w542]
      tunnel: w245 -> [w258 _ _ _ _ _ _ _ _ _ _ _ _ _ _ _ _ _ _]
      event Timeout {
        n136 = event-data() -> ()  [unwired: 1 in, 1 out]
        n137 = local read "Mode"() -> (w263:T3)
        n138 = case shown="\"Commands\"" "Dashboard Tab" {
          tunnel: w266 -> [_ _ w282 _ _]
          tunnel: "TestMode/Automatic/" ("Name Pattern") -> [_ _ w281 _ _]
          tunnel: T19 [{"Operation"=enum."Clear", "Color Box"=14013909}, {"Operation"=enum."Clear", "Color Box"=14013909}, {"Operation"=enum."Clear", "Color Box"=14013909}, {"Operation"=enum."Clear", "Color Box"=14013909}, {"Operation"=enum."Update", "Color Box"=14013909}, {"Operation"=enum."Update", "Color Box"=16777215}, {"Operation"=enum."Clear", "Color Box"=14013909}, {"Operation"=enum."Clear", "Color Box"=14013909}, {"Operation"=enum."Clear", "Color Box"=14013909}] -> [_ _ w274 _ w302]
          tunnel: w263 -> [_ _ w273 _ w301]
          tunnel: u32[] [15790320, 15790320, 15790320, 15790320, 16777215, 16777215, 15790320, 15790320, 15790320] -> [_ _ _ _ w307]
          tunnel: w261 -> [_ _ _ _ w295]
          tunnel: w258 -> [_ w268 _ _ _]
          frame "Custom", Default {
          }
          frame "Basic" {
            n139 = call <vilib>:"WPI_DashboardUpdateNames.vi"("Controls on Tab"=w268) -> ()  [unwired: 11 in]
          }
          frame "Test" {
            w280 = -2 ("Active Item:Row Number")
            n140 = Index Array(array=w274, index=w273) -> (element=w275:T22)
            n141 = Unbundle(w275) -> ("Operation"=w276:enum16{"Update", "Clear"}, "Color Box"=w277:u32)
            n142 = call <vilib>:"NT Read String.vi"("Name"="TestMode/TestName") -> ("String"=w271:string)  [unwired: 9 in, 1 out]
            n143 = call <vilib>:"NT Read and Format Entries as Tree.vi"("Operation"=w276, "Name Pattern"=w281, "Tree Refnum"=w282) -> ()  [unwired: 7 in, 2 out]
            n144 = case shown="\"\"" w271 {
              tunnel: "TestMode/TestProgress" ("Name") -> [w284 _]
              tunnel: "TestMode/TestProgressText" ("Name") -> [w283 _]
              frame Default {
                n145 = call <vilib>:"NT Read Number.vi"("Name"=w284) -> ("Numeric"=w285:dbl)  [unwired: 9 in, 1 out]
                n146 = call <vilib>:"NT Read String.vi"("Name"=w283) -> ("String"=w286:string)  [unwired: 9 in, 1 out]
                n147 = Bundle("Numeric"=w285, "String"=w286) -> (→"Progress":cluster{"Numeric":dbl, "String":string})  [unwired: 1 in]
              }
              frame "" {
                n148 = property on="Progress" class="Clust (strict)"("Visible"=FALSE) -> ()  [unwired: 2 in, 2 out]
                n149 = local write "Test Name"(u16 0) -> ()
              }
            }
            n150 = property on="Test Tree" class="Tree (strict)"("Active Item Row Number"=w280, "ActiveColNum"=w280, "CellBG"=w277, "Active Item Row Number"=-1 ("Active Item:Row Number"), "CellBG"=u32 5789784 ("Color Box")) -> ()  [unwired: 2 in, 2 out]
          }
          frame "Variables" {
            w292 = string[] ["CameraPublisher", "Usage", "DB"]  # Items to initially close
            n151 = First Call?() -> (First Call?: T/F=w293:bool)
            n152 = control-ref of="Tree"() -> (w294:refnum<vi>)
            n153 = Select(t=w292, s=w293, f=string[] []) -> (s? t:f=w290:string[])
            n154 = call <vilib>:"NT Read and Format Entries as Tree.vi"("Tags to  Close"=w290, "Tree Refnum"=w294) -> ()  [unwired: 8 in, 2 out]
          }
          frame "Commands" {
            w303 = u32 5789784 ("Color Box")
            w304 = T23 {"Row"=-1, "Column"=-2} ("Active Cell:Active Cell")
            w306 = T23 {"Row"=-2, "Column"=-2} ("Active Cell:Active Cell")
            n155 = Index Array(array=w307, index=w301) -> (element=w305:u32)
            n156 = Index Array(array=w302, index=w301) -> (element=w300:T22)
            n157 = Unbundle(w300) -> ("Operation"=w299:enum16{"Update", "Clear"})  [unwired: 1 out]
            n158 = local read "Command Selection"() -> (w298:i32)
            n159 = property on="Command Selection" class="MCListbox (strict)"("ActiveCell"=w306, "CellBG"=w305, "ActiveCell"=w304, "CellBG"=w303) -> ()  [unwired: 2 in, 2 out]
            n160 = call <vilib>:"WPI_DashboardUpdate RPC Info.vi"("Operation"=w299) -> ("update"=w297:bool, "commands"=w296:string[][])  [unwired: 9 in]
            n161 = property on="Command Selection" class="MCListbox (strict)"("ItemNames"=w296) -> ()  [unwired: 2 in, 2 out]
            n162 = property on="Command Params" class="Tbl (strict)"("Active Cell"=w306, "Cell BG Color"=w305, "Active Cell"=w304, "Cell BG Color"=w303) -> ()  [unwired: 2 in, 2 out]
            n163 = call <vilib>:"WPI_DashboardUpdate Command Params.vi"("Update"=w297, "NewVal"=w298, "Commands"=w296, "Param Tbl"=w295) -> ()  [unwired: 7 in, 1 out]
          }
        }
        n164 = call <vilib>:"Connextion Info.vi"() -> ("Connected"=→"NT Connection":bool)  [unwired: 10 in, 1 out]
      }
      event "Test Tree": Value Change {
        # "Show appropriate\ncontrols"
        n165 = event-data() -> ("CtlRef"=w312:refnum<vi>, "NewVal"=w310:string)  [unwired: 1 in]
        n166 = call <vilib>:"WPI_UtilitiesGetTreeIOName.vi"("NewVal"=w310, "TreeControl in"=w312) -> ("I/O Name"=w313:string)  [unwired: 9 in]
        n167 = case shown="\"Camera\"" w313 {
          selector: w313 -> [_ w320 _ w342 w351 _]
          tunnel: w310 -> [_ _ w339 w341 _ w358]
          tunnel: cluster{string[]}[] [{["640x480", "320x240", "160x120"]}, {["Auto", "Fixed indoor", "Fixed outdoor 1", "Fixed outdoor 2", "Fixed fluorescent 1", "Fixed fluorescent 2", "Hold current"]}, {["Auto", "Flicker-free 50 Hz", "Flicker-free 60 Hz", "Hold current"]}, {["None", "Prioritize frame rate", "Prioritize image quality"]}, {["Monochrome", "Color"]}] -> [_ _ _ _ _ w357]
          frame Default {
            w315 = FALSE ("Visible")
            w314 = FALSE ("Visible")
            n168 = property on="Motor" class="Clust (strict)"("Visible"=w314) -> ()  [unwired: 2 in, 2 out]
            n169 = property on="Test Ring" class="Ring (strict)"("Visible"=w314) -> ()  [unwired: 2 in, 2 out]
            n170 = property on="Rev/Fwd" class="Clust (strict)"("Visible"=w315) -> ()  [unwired: 2 in, 2 out]
            n171 = property on="On/Off" class="Bool (strict)"("Visible"=w315) -> ()  [unwired: 2 in, 2 out]
            n172 = property on="Test Slider" class="Slide (strict)"("Visible"=w315) -> ()  [unwired: 2 in, 2 out]
          }
          frame "Analog Out", "Motor", "PWM" {
            w321 = FALSE ("Visible")
            n173 = case shown="\"Analog Out\"" w320 {
              tunnel: [1.0 ("Value") -1.0 ("Value") 0.0 ("Value")] -> w319
              tunnel: [255.0 ("Value") 1.0 ("Value") 5.0 ("Value")] -> w318
              tunnel: [128.0 ("Value") 0.0 ("Value") 0.0 ("Value")] -> w317
              tunnel: [64.0 ("Value") 0.5 ("Value") 1.0 ("Value")] -> w316
              frame "PWM" {
              }
              frame "Motor", Default {
              }
              frame "Analog Out" {
              }
            }
            n174 = property on="Motor" class="Clust (strict)"("Visible"=TRUE) -> ()  [unwired: 2 in, 2 out]
            n175 = property on="Value" class="Slide (strict)"("Value"=w317, "Scale.Minimum"=w319, "Scale.Maximum"=w318, "Scale.Increment"=w316) -> ()  [unwired: 2 in, 2 out]
            n176 = property on="On/Off" class="Bool (strict)"("Visible"=w321) -> ()  [unwired: 2 in, 2 out]
            n177 = property on="Test Slider" class="Slide (strict)"("Visible"=w321) -> ()  [unwired: 2 in, 2 out]
            n178 = property on="Test Ring" class="Ring (strict)"("Visible"=w321) -> ()  [unwired: 2 in, 2 out]
            n179 = property on="Rev/Fwd" class="Clust (strict)"("Visible"=w321) -> ()  [unwired: 2 in, 2 out]
          }
          frame "Servo" {
            w337 = FALSE ("Visible")
            n180 = call <vilib>:"NT Read Number.vi"("Name"=w339) -> ("Numeric"=w338:dbl)  [unwired: 9 in, 1 out]
            n181 = property on="Test Slider" class="Slide (strict)"("Visible"=TRUE, "Scale.Maximum"=170.0 ("Scale.Range:Maximum")) -> ()  [unwired: 2 in, 2 out]
            n182 = local write "Test Slider"(w338) -> ()
            n183 = property on="Motor" class="Clust (strict)"("Visible"=w337) -> ()  [unwired: 2 in, 2 out]
            n184 = property on="Rev/Fwd" class="Clust (strict)"("Visible"=w337) -> ()  [unwired: 2 in, 2 out]
            n185 = property on="On/Off" class="Bool (strict)"("Visible"=w337) -> ()  [unwired: 2 in, 2 out]
            n186 = property on="Test Ring" class="Ring (strict)"("Visible"=w337) -> ()  [unwired: 2 in, 2 out]
          }
          frame "Relay", "Solenoid" {
            w340 = FALSE ("Visible")
            n187 = property on="Motor" class="Clust (strict)"("Visible"=w340) -> ()  [unwired: 2 in, 2 out]
            n188 = property on="Test Slider" class="Slide (strict)"("Visible"=w340) -> ()  [unwired: 2 in, 2 out]
            n189 = Search and Replace String(input string=w341, search string="/Value  **", replace string="/Direction") -> (result string=w347:string)  [unwired: 5 in, 3 out]
            n190 = property on="Test Ring" class="Ring (strict)"("Visible"=w340) -> ()  [unwired: 2 in, 2 out]
            n191 = call <vilib>:"NT Read String.vi"("Name"=w347) -> ("String"=w345:string)  [unwired: 9 in, 1 out]
            n192 = Equal?(x="Both directions", y=w345) -> (x = y?=w343:bool)
            n193 = Not(x=w343) -> (.not. x?=w344:bool)
            n194 = property on="Rev/Fwd" class="Clust (strict)"("Visible"=w343) -> ()  [unwired: 2 in, 2 out]
            n195 = property on="On/Off" class="Bool (strict)"("Visible"=w344, "Caption.Text"=w342) -> ()  [unwired: 2 in, 2 out]
          }
          frame "Compressor", "Digital Out" {
            w350 = FALSE ("Visible")
            # "Get direction and finish"
            n196 = property on="Motor" class="Clust (strict)"("Visible"=w350) -> ()  [unwired: 2 in, 2 out]
            n197 = property on="Test Slider" class="Slide (strict)"("Visible"=w350) -> ()  [unwired: 2 in, 2 out]
            n198 = property on="Test Ring" class="Ring (strict)"("Visible"=w350) -> ()  [unwired: 2 in, 2 out]
            n199 = property on="On/Off" class="Bool (strict)"("Visible"=TRUE, "Caption.Text"=w351) -> ()  [unwired: 2 in, 2 out]
            n200 = property on="Rev/Fwd" class="Clust (strict)"("Visible"=FALSE) -> ()  [unwired: 2 in, 2 out]
          }
          frame "Camera" {
            n201 = call <vilib>:"Get Last Path Segment.vi"("String in"=w358) -> ("String out"=w359:string)  [unwired: 10 in]
            n202 = property on="On/Off" class="Bool (strict)"("Visible"=FALSE) -> ()  [unwired: 2 in, 2 out]
            n203 = property on="Motor" class="Clust (strict)"("Visible"=FALSE) -> ()  [unwired: 2 in, 2 out]
            n204 = property on="Rev/Fwd" class="Clust (strict)"("Visible"=FALSE) -> ()  [unwired: 2 in, 2 out]
            n205 = case shown="\"White Balance  **\"" w359 {
              tunnel: w358 -> [w365 w374 w383 w392 w401 _ w407]
              tunnel: w357 -> [w363 w371 w380 w389 w398 _ _]
              frame "Size  **" {
                n206 = Index Array(array=w363) -> (element=w362:cluster{string[]})  [unwired: 1 in]
                n207 = call <vilib>:"NT Read String.vi"("Name"=w365) -> ("String"=w364:string)  [unwired: 9 in, 1 out]
                n208 = Unbundle(w362) -> (w360:string[])
                n209 = Match First String(2:w360, 3:w364) -> (0:w361:i32)  [unwired: 1 out]
                n210 = property on="Test Ring" class="Ring (strict)"("Value"=w361, "Strings []"=w360) -> ()  [unwired: 2 in, 2 out]
                n211 = property on="Test Ring" class="Ring (strict)"("Visible"=TRUE) -> ()  [unwired: 2 in, 2 out]
                n212 = property on="Test Slider" class="Slide (strict)"("Visible"=FALSE) -> ()  [unwired: 2 in, 2 out]
              }
              frame "White Balance  **" {
                n213 = Index Array(array=w371, index=1) -> (element=w372:cluster{string[]})
                n214 = call <vilib>:"NT Read String.vi"("Name"=w374) -> ("String"=w373:string)  [unwired: 9 in, 1 out]
                n215 = Unbundle(w372) -> (w369:string[])
                n216 = Match First String(2:w369, 3:w373) -> (0:w368:i32)  [unwired: 1 out]
                n217 = property on="Test Ring" class="Ring (strict)"("Value"=w368, "Strings []"=w369) -> ()  [unwired: 2 in, 2 out]
                n218 = property on="Test Ring" class="Ring (strict)"("Visible"=TRUE) -> ()  [unwired: 2 in, 2 out]
                n219 = property on="Test Slider" class="Slide (strict)"("Visible"=FALSE) -> ()  [unwired: 2 in, 2 out]
              }
              frame "Exposure  **" {
                n220 = Index Array(array=w380, index=2) -> (element=w381:cluster{string[]})
                n221 = call <vilib>:"NT Read String.vi"("Name"=w383) -> ("String"=w382:string)  [unwired: 9 in, 1 out]
                n222 = Unbundle(w381) -> (w377:string[])
                n223 = Match First String(2:w377, 3:w382) -> (0:w378:i32)  [unwired: 1 out]
                n224 = property on="Test Ring" class="Ring (strict)"("Value"=w378, "Strings []"=w377) -> ()  [unwired: 2 in, 2 out]
                n225 = property on="Test Ring" class="Ring (strict)"("Visible"=TRUE) -> ()  [unwired: 2 in, 2 out]
                n226 = property on="Test Slider" class="Slide (strict)"("Visible"=FALSE) -> ()  [unwired: 2 in, 2 out]
              }
              frame "Exposure Priority  **" {
                n227 = Index Array(array=w389, index=3) -> (element=w390:cluster{string[]})
                n228 = call <vilib>:"NT Read String.vi"("Name"=w392) -> ("String"=w391:string)  [unwired: 9 in, 1 out]
                n229 = Unbundle(w390) -> (w386:string[])
                n230 = Match First String(2:w386, 3:w391) -> (0:w387:i32)  [unwired: 1 out]
                n231 = property on="Test Ring" class="Ring (strict)"("Value"=w387, "Strings []"=w386) -> ()  [unwired: 2 in, 2 out]
                n232 = property on="Test Ring" class="Ring (strict)"("Visible"=TRUE) -> ()  [unwired: 2 in, 2 out]
                n233 = property on="Test Slider" class="Slide (strict)"("Visible"=FALSE) -> ()  [unwired: 2 in, 2 out]
              }
              frame "Color Enable  **" {
                n234 = Index Array(array=w398, index=4) -> (element=w399:cluster{string[]})
                n235 = call <vilib>:"NT Read String.vi"("Name"=w401) -> ("String"=w400:string)  [unwired: 9 in, 1 out]
                n236 = Unbundle(w399) -> (w395:string[])
                n237 = Match First String(2:w395, 3:w400) -> (0:w396:i32)  [unwired: 1 out]
                n238 = property on="Test Ring" class="Ring (strict)"("Value"=w396, "Strings []"=w395) -> ()  [unwired: 2 in, 2 out]
                n239 = property on="Test Ring" class="Ring (strict)"("Visible"=TRUE) -> ()  [unwired: 2 in, 2 out]
                n240 = property on="Test Slider" class="Slide (strict)"("Visible"=FALSE) -> ()  [unwired: 2 in, 2 out]
              }
              frame Default {
                n241 = property on="Test Ring" class="Ring (strict)"("Visible"=FALSE) -> ()  [unwired: 2 in, 2 out]
                n242 = property on="Test Slider" class="Slide (strict)"("Visible"=FALSE) -> ()  [unwired: 2 in, 2 out]
              }
              frame "Brightness  **", "Color Level  **", "Compression  **", "FPS  **", "Sharpness  **" {
                n243 = call <vilib>:"NT Read Number.vi"("Name"=w407) -> ("Numeric"=w406:dbl)  [unwired: 9 in, 1 out]
                n244 = local write "Test Slider"(w406) -> ()
                n245 = property on="Test Slider" class="Slide (strict)"("Visible"=TRUE, "Scale.Maximum"=100.0 ("Scale.Range:Maximum")) -> ()  [unwired: 2 in, 2 out]
                n246 = property on="Test Ring" class="Ring (strict)"("Visible"=FALSE) -> ()  [unwired: 2 in, 2 out]
              }
            }
          }
        }
        n247 = property on="Progress" class="Clust (strict)"("Visible"=FALSE) -> ()  [unwired: 2 in, 2 out]
      }
      event "Test Name": Mouse Enter {
        # "Populate the ring with the list of tests"
        n248 = event-data() -> ()  [unwired: 1 in, 1 out]
        n249 = call <vilib>:"NT Read String Array.vi"("Name"="TestMode/TestList") -> ("String Array"=w415:string[])  [unwired: 9 in, 1 out]
        n250 = Build Array (concatenate)("Select the test to run...", w415) -> (w414:string[])
        n251 = property on="Test Name" class="Ring (strict)"("Strings []"=w414) -> ()  [unwired: 2 in, 2 out]
      }
      event "Test Name": Value Change {
        w417 = FALSE ("Visible")
        # "Tell the robot the test name to run"
        n252 = event-data() -> ("NewVal"=w421:u16)  [unwired: 1 in]
        n253 = property on="Test Name" class="Ring (strict)"() -> ("Strings []"=w422:string[])  [unwired: 2 in, 2 out]
        n254 = local write "Progress"(T5 {"Test Progress"=0, "Test Progress Text"=""} ("Progress")) -> ()
        n255 = Index Array(array=w422, index=w421) -> (element=w420:string)
        n256 = call <vilib>:"NT Write String.vi"("String"=w420, "Name"="TestMode/TestName") -> ()  [unwired: 9 in, 1 out]
        n257 = property on="Progress" class="Clust (strict)"("Visible"=TRUE) -> ()  [unwired: 2 in, 2 out]
        n258 = property on="Motor" class="Clust (strict)"("Visible"=w417) -> ()  [unwired: 2 in, 2 out]
        n259 = property on="Test Slider" class="Slide (strict)"("Visible"=w417) -> ()  [unwired: 2 in, 2 out]
        n260 = property on="On/Off" class="Bool (strict)"("Visible"=w417) -> ()  [unwired: 2 in, 2 out]
        n261 = property on="Rev/Fwd" class="Clust (strict)"("Visible"=w417) -> ()  [unwired: 2 in, 2 out]
        n262 = property on="Test Ring" class="Ring (strict)"("Visible"=w417) -> ()  [unwired: 2 in, 2 out]
      }
      event "Command Selection": Value Change {
        # "Get the params and show in table"
        n263 = event-data() -> ("NewVal"=w427:i32)  [unwired: 1 in]
        n264 = property on="Command Selection" class="MCListbox (strict)"() -> ("ItemNames"=w425:string[][])  [unwired: 2 in, 2 out]
        n265 = call <vilib>:"WPI_DashboardUpdate Command Params.vi"("NewVal"=w427, "Commands"=w425, "Param Tbl"=w426) -> ()  [unwired: 8 in, 1 out]
      }
      event "Execute Command": Value Change {
        # "Started one, Unique ID holds\nresponse"
        n266 = event-data() -> ()  [unwired: 1 in, 1 out]
        n267 = property on="Command Selection" class="MCListbox (strict)"() -> ("ItemNames"=w438:string[][])  [unwired: 2 in, 2 out]
        n268 = Index Array(array=w438, index (row)="Command Selection", index (col)=0) -> (element=w436:string)
        n269 = call <vilib>:"Invoke Commands.vi"("Command Params"="Command Params", "Function Name"=w436) -> ("Params"=w432:u8, "Started"=w431:bool)  [unwired: 7 in, 1 out]
        n270 = Array Subset(array="Command Params", length (row)=w432) -> (w433:string[][])  [unwired: 3 in]
        n271 = Select(t="Executing" ("Cmd Status"), s=w431, f="" ("Cmd Status")) -> (s? t:f=→"Cmd Status":string)
      }
      event "Command Selection": Double Click {
        n272 = event-data() -> ("Row"=w446:i32)  [unwired: 1 in]
        n273 = property on="Command Selection" class="MCListbox (strict)"() -> ("ItemNames"=w449:string[][])  [unwired: 2 in, 2 out]
        n274 = local read "Command Params"() -> (w445:string[][])
        n275 = Index Array(array=w449, index (row)=w446, index (col)=0) -> (element=w447:string)
        n276 = call <vilib>:"Invoke Commands.vi"("Command Params"=w445, "Function Name"=w447) -> ("Params"=w444:u8, "Started"=w439:bool)  [unwired: 7 in, 1 out]
        n277 = Array Subset(array=w445, length (row)=w444) -> (w443:string[][])  [unwired: 3 in]
        n278 = Select(t="Executing" ("Cmd Status"), s=w439, f="" ("Cmd Status")) -> (s? t:f=w440:string)
        n279 = local write "Cmd Status"(w440) -> ()
      }
      event "CheckList": Double Click {
        # "Shift clears all"
        # "Update symbols on the listbox"
        n280 = event-data() -> ("PlatMods.Shift"=w451:bool, "Row"=w453:i32)  [unwired: 1 in]
        n281 = case shown="True" w451 {
          tunnel: w453 -> [w457 _]
          tunnel: 1 -> [w456 _]
          frame False {
            n282 = property on="CheckList" class="LstBox (strict)"() -> ("Item Symbols"=w455:i32[])  [unwired: 2 in, 2 out]
            n283 = Replace Array Subset(array=w455, new element=w456, index=w457) -> (w454:i32[])
            n284 = property on="CheckList" class="LstBox (strict)"("Item Symbols"=w454) -> ()  [unwired: 2 in, 2 out]
          }
          frame True {
            w458 = 0 ("Top Row")
            n285 = property on="CheckList" class="LstBox (strict)"() -> ("Number of Rows"=w460:u32)  [unwired: 2 in, 2 out]
            n286 = Initialize Array(0, w460) -> (w459:i32[])
            n287 = property on="CheckList" class="LstBox (strict)"("Top Row"=w458, "Value"=w458, "Item Symbols"=w459) -> ()  [unwired: 2 in, 2 out]
          }
        }
      }
      event "CheckList": Key Down {
        # "Update symbols on the listbox\nLeft and right keys check and uncheck"
        n288 = event-data() -> ("VKey"=w464:T20)  [unwired: 1 in]
        n289 = case shown="\"Left\", \"Right\"" w464 {
          selector: w464 -> [w469 _]
          tunnel: eventvkey."Left" ("VKey") -> [w467 _]
          frame "Left", "Right" {
            n290 = Equal?(x=w467, y=w469) -> (x = y?=w468:bool)
            n291 = Select(t=0, s=w468, f=1) -> (s? t:f=w470:i32)
            n292 = property on="CheckList" class="LstBox (strict)"() -> ("Item Symbols"=w473:i32[])  [unwired: 2 in, 2 out]
            n293 = Replace Array Subset(array=w473, new element=w470, index="CheckList") -> (w472:i32[])
            n294 = property on="CheckList" class="LstBox (strict)"("Item Symbols"=w472) -> ()  [unwired: 2 in, 2 out]
          }
          frame Default {
          }
        }
      }
      event "Motor.Enable": Value Change {
        # "When the test mode otor enable helper is set, update that\ntree row item's value"
        n295 = event-data() -> ("NewVal"=w479:bool)  [unwired: 1 in]
        n296 = Unbundle("Motor") -> ("Value"=w478:dbl)  [unwired: 1 out]
        n297 = Select(t=w478, s=w479, f=0.0) -> (s? t:f=w476:dbl)
        n298 = call <vilib>:"NT Write Number.vi"("Numeric"=w476, "Name"=w475) -> ()  [unwired: 9 in, 1 out]
      }
      event "Test Slider": Value Change {
        # "When the test mode slider helper is set, update that\ntree row item's value"
        n299 = event-data() -> ("NewVal"=w482:dbl)  [unwired: 1 in]
        n300 = call <vilib>:"NT Write Number.vi"("Numeric"=w482, "Name"=w483) -> ()  [unwired: 9 in, 1 out]
      }
      event "On/Off": Value Change {
        # "When the test mode on/off helper value is set, update that\ntree row item's value"
        n301 = event-data() -> ("NewVal"=w487:bool)  [unwired: 1 in]
        n302 = Boolean To (0,1)(Boolean=w487) -> (0, 1=w486:i16)
        n303 = call <vilib>:"NT Write Number.vi"("Numeric"=w486, "Name"=w485) -> ()  [unwired: 9 in, 1 out]
      }
      event "Rev/Fwd": Value Change {
        # "When the test mode helper value for relays is set, update that\ntree row item's value"
        n304 = event-data() -> ("NewVal.Forward"=w495:bool, "NewVal.Reverse"=w494:bool)  [unwired: 1 in]
        n305 = Boolean To (0,1)(Boolean=w495) -> (0, 1=w491:i16)
        n306 = Boolean To (0,1)(Boolean=w494) -> (0, 1=w493:i16)
        n307 = Negate(x=w493) -> (-x=w492:i16)
        n308 = Add(x=w491, y=w492) -> (x+y=w490:i16)
        n309 = call <vilib>:"NT Write Number.vi"("Numeric"=w490, "Name"=w489) -> ()  [unwired: 9 in, 1 out]
      }
      event "Test Ring": Value Change {
        # "When a test mode helper value is selected from the ring,\nset the tree item's variable to the string value"
        n310 = event-data() -> ("NewVal"=w499:u16)  [unwired: 1 in]
        n311 = property on="Test Ring" class="Ring (strict)"() -> ("Strings []"=w500:string[])  [unwired: 2 in, 2 out]
        n312 = Index Array(array=w500, index=w499) -> (element=w498:string)
        n313 = call <vilib>:"NT Write String.vi"("String"=w498, "Name"=w497) -> ()  [unwired: 9 in, 1 out]
      }
      event "Rec Mode": Value Change {
        # "Update globals for recording mode and path to read log from.\nClear when logging and let NetworkTables set path for vision to\nuse."
        n314 = event-data() -> ("NewVal"=w511:enum32{"Stop", "Record", "Playback"})  [unwired: 1 in]
        n315 = global write "WPI_DashboardLogging Global.vi" "Logging Filename"(path "") -> ()
        n316 = global write "WPI_DashboardLogging Global.vi" "Recording"(w511) -> ()
        n317 = case shown="\"Playback\"" w511 {
          tunnel: w510 -> [_ w513 w522]
          tunnel: [_ _ w521] -> w508
          tunnel: [_ _ w520] -> _
          tunnel: w506 -> [_ _ w518]
          tunnel: cluster{i32, i32} {-250, 170} -> [_ _ w517]
          tunnel: [_ _ T21 {"Image Size"=TRUE, "Image Type"=TRUE, "Pixel Value"=TRUE, "ROI Information"=TRUE, "Zoom Factor"=FALSE} ("Image Information Shown:All Elements")] -> w501
          tunnel: [_ _ TRUE ("Zoom Factor")] -> w502
          tunnel: w504 -> [_ _ w514]
          frame Default {
          }
          frame "Stop", "Record" {
            # "Place Window too"
            n318 = invoke class="VI" method="FP.Close"(reference=w513) -> (reference out=w512:refnum<vi>)  [unwired: 2 in, 2 out]
            n319 = invoke class="VI" method="Abort VI"(reference=w512) -> ()  [unwired: 2 in, 3 out]
          }
          frame "Playback" {
            n320 = call "Open Playback Panel.vi"("Offset"=w517, "DB VI Ref"=w518, "Playback in"=w522) -> ("Playback out"=w519:refnum<vi>)  [unwired: 8 in]
            n321 = register-events(w519, w514) -> (reference out=w521:refnum<event-registration>, error out=w520:errorcluster)  [unwired: 2 in]
          }
        }
        n322 = property on="Camera Image Right" class="ImageControl"("Image Information Shown"=w501, "Image Information Visible"=w502) -> ()  [unwired: 2 in, 2 out]
        n323 = property on="Camera Image" class="ImageControl"("Image Information Shown"=w501, "Image Information Visible"=w502) -> ()  [unwired: 2 in, 2 out]
        n324 = call <vilib>:"WPI_DashboardNT Log FieldName Cache.vi"("Operation"=enum16{"Lookup/Add", "Index", "Clear"}."Clear") -> ()  [unwired: 8 in, 3 out]
      }
      event Panel Close {
        w524 = enum32{"Stop", "Record", "Playback"}."Stop" ("Rec Mode")
        # "Playback window has been closed, abort"
        n325 = event-data() -> ()  [unwired: 1 in, 4 out]
        n326 = local write "Rec Mode"(w524) -> ()
        n327 = global write "WPI_DashboardLogging Global.vi" "Recording"(w524) -> ()
      }
      event Panel Close {
        # "Abort playback window and ourself"
        n328 = event-data() -> ()  [unwired: 1 in, 4 out]
        n329 = invoke class="VI" method="FP.Close"(reference=w528) -> (reference out=w527:refnum<vi>)  [unwired: 2 in, 2 out]
        n330 = invoke class="VI" method="Abort VI"(reference=w527) -> (error out=w526:errorcluster)  [unwired: 2 in, 2 out]
        n331 = invoke class="VI" method="Abort VI"(error in=w526) -> ()  [unwired: 2 in, 3 out]
      }
      event User Event {
        n332 = event-data() -> ("IDs"=w535:cluster{"RPC field ID":u16, "Unique ID":u16}, "String"=w534:string)  [unwired: 1 in]
        n333 = Bundle("IDs"=w535, "String"=w534) -> (w533:T8)  [unwired: 1 in]
        n334 = call <vilib>:"Retrieve RPC Response.vi"("RPC Response"=w533) -> ("Output"=w531:string[][])  [unwired: 10 in]
        n335 = Build Array (concatenate)(w529, w531) -> (w530:string[][])
        n336 = local write "Command Params"(w530) -> ()
        n337 = local write "Cmd Status"("" ("Cmd Status")) -> ()
      }
      event "Tree": Double Click {
        n338 = event-data() -> ("PlatMods"=w541:T24, "Tag"=w538:string)  [unwired: 1 in]
        n339 = Unbundle(w541) -> ("Shift"=w540:bool)  [unwired: 4 out]
        n340 = String Subset(string=w538, length (rest)=1 ("length (rest)")) -> (substring=w537:string)  [unwired: 1 in]
        n341 = Not(x=w540) -> (.not. x?=w539:bool)
        n342 = case shown="\"/\"" w537 {
          tunnel: w538 -> [_ w544]
          tunnel: w539 -> [_ w543]
          frame Default {
          }
          frame "/" {
            n343 = call <vilib>:"NT Update Persistence.vi"("Persistence"=w543, "Name"=w544) -> ()  [unwired: 9 in, 1 out]
          }
        }
      }
    }
  }
  n344 = while {
    tunnel: w62 -> [w546]
    i -> [w549]
    stop <- FALSE stop-if-true
    n345 = Wait (ms)(milliseconds to wait=u32 100) -> ()  [unwired: 1 out]
    n346 = case shown="\"Playback\"" "Rec Mode" {
      tunnel: w549 -> [_ _ w564]
      tunnel: [u32 2829099 ("Base Color") u32 11141120 ("Target Color") w553] -> w545
      frame "Stop", Default {
        # "Reset the color, extra updates don't cost much"
      }
      frame "Record" {
      }
      frame "Playback" {
        # "Playback"
        n347 = Quotient & Remainder(x=w564, y=u32 50 ("milliseconds to wait")) -> (x-y*floor(x/y)=w560:u32)  [unwired: 1 out]
        n348 = Divide(x=w560, y=u32 50 ("milliseconds to wait")) -> (x/y=w557:dbl)
        n349 = Multiply(x=6.283185307179586, y=w557) -> (x*y=w562:dbl)
        n350 = Sine(x=w562) -> (sin(x)=w561:dbl)
        n351 = Absolute Value(x=w561) -> (abs(x)=w554:dbl)
        n352 = call "Interpolate RGB Color.vi"("Proportion"=w554, "Target Color"=u32 30976, "Base Color"=u32 2829099) -> ("Result Color"=w553:u32)  [unwired: 8 in]
      }
    }
    n353 = property class="Pane"(reference=w546, "PaneColor"=w545) -> ()  [unwired: 1 in, 2 out]
  }
  n354 = local write "Dashboard Tab"(T2."Drive" ("Dashboard Tab")) -> ()
  n355 = property on="On/Off" class="Bool (strict)"("Visible"=w34) -> ()  [unwired: 2 in, 2 out]
  n356 = property on="Motor" class="Clust (strict)"("Visible"=w34) -> ()  [unwired: 2 in, 2 out]
  n357 = property on="Progress" class="Clust (strict)"("Visible"=w34) -> ()  [unwired: 2 in, 2 out]
  n358 = property on="Test Ring" class="Ring (strict)"("Visible"=w34) -> ()  [unwired: 2 in, 2 out]
  n359 = property on="Rev/Fwd" class="Clust (strict)"("Visible"=w34) -> ()  [unwired: 2 in, 2 out]
  n360 = while {
    tunnel: u16 1741 ("timeout ms (25000)") -> [w566]
    stop <- FALSE stop-if-true
    n361 = TCP Create Listener(10:w566) -> (0:w565:errorcluster, 3:w567:refnum<k5>)  [unwired: 4 in, 1 out]
    n362 = case shown="No Error" w565 {
      selector: w565 -> [w569 _]
      tunnel: w567 -> [w570 _]
      frame No Error {
        n363 = while {
          tunnel: w570 -> [w573]
          tunnel: w569 -> [w572]
          stop <- FALSE stop-if-true
          n364 = TCP Wait On Listener(8:w572, 11:w573) -> (0:w574:errorcluster, 4:w575:refnum<k5>)  [unwired: 2 in, 3 out]
          n365 = local write "TCP"(w575) -> ()
          n366 = case shown="No Error" w574 {
            frame No Error {
            }
            frame Error {
              n367 = Wait (ms)(milliseconds to wait=u32 1000) -> ()  [unwired: 1 out]
            }
          }
        }
      }
      frame Error {
        n368 = Wait (ms)(milliseconds to wait=u32 1000) -> ()  [unwired: 1 out]
      }
    }
  }
  n369 = local write "Command Selection"(u16 0 ("milliseconds to wait")) -> ()
  n370 = local write "Command Params"(string[][] [] ("Command Params")) -> ()
  n371 = global write "WPI_DashboardLogging Global.vi" "Recording"(w56) -> ()
  n372 = local write "Rec Mode"(w56) -> ()
  n373 = while {
    stop <- FALSE stop-if-true
    n374 = call-poly <vilib>:"NT Read Value.vi"("Name"="PixyX") -> ("Numeric"=→"PixyX":dbl)  [unwired: 9 in, 1 out]
    n375 = call-poly <vilib>:"NT Read Value.vi"("Name"="Gyro") -> ("Numeric"=→"Gyro":dbl)  [unwired: 9 in, 1 out]
    n376 = call-poly <vilib>:"NT Read Value.vi"("Name"="Ultrasonic") -> ("Numeric"=→"Ultrasonic":dbl)  [unwired: 9 in, 1 out]
    n377 = call-poly <vilib>:"NT Read Value.vi"("Name"="Elevator") -> ("Numeric"=→"Elevator":dbl)  [unwired: 9 in, 1 out]
    n378 = call-poly <vilib>:"NT Read Value.vi"("Name"="LeftEncoder") -> ("Numeric"=→"LeftEncoder":dbl)  [unwired: 9 in, 1 out]
    n379 = call-poly <vilib>:"NT Read Value.vi"("Name"="RightEncoder") -> ("Numeric"=→"RightEncoder":dbl)  [unwired: 9 in, 1 out]
    n380 = call-poly <vilib>:"NT Read Value.vi"("Name"="TopLimit") -> ("Boolean"=→"Top":bool)  [unwired: 9 in, 1 out]
    n381 = call-poly <vilib>:"NT Write Value.vi"("Boolean"="Reset", "Name"="Reset") -> ()  [unwired: 9 in, 1 out]
    n382 = call-poly <vilib>:"NT Read Value.vi"("Name"="BottomLimit") -> ("Boolean"=→"Bottom":bool)  [unwired: 9 in, 1 out]
    n383 = call-poly <vilib>:"NT Read Value.vi"("Name"="SlowMode") -> ("Boolean"=w583:bool)  [unwired: 9 in, 1 out]
    n384 = Not(x=w583) -> (.not. x?=→"FastMode":bool)
    n385 = call-poly <vilib>:"NT Read Value.vi"("Name"="ToggleMode") -> ("Boolean"=→"ToggleMode":bool)  [unwired: 9 in, 1 out]
    n386 = call-poly <vilib>:"NT Read Value.vi"("Name"="HasCube") -> ("Boolean"=→"HasCube":bool)  [unwired: 9 in, 1 out]
    n387 = Wait (ms)(milliseconds to wait=u32 80) -> ()  [unwired: 1 out]
  }
